vi "Rule_Check_Win.vi"(8 "error in":errorcluster, 9 "Exact Five":bool, 10 "Last Move":T2={"Row"=7, "Col"=7, "Stone"=enum."Black"}, 11 "Grid":enum8{"Empty", "Black", "White"}[][](array[ring])=[[enum."Empty", enum."Empty", enum."Empty", enum."Empty", enum."Empty", enum."Empty", enum."Empty", enum."Empty", enum."Empty", enum."Empty", enum."Empty", enum."Empty", enum."Empty", enum."Empty", enum."Empty"], [enum."Empty", enum."Empty", enum."Empty", enum."Empty", enum."Empty", enum."Empty", enum."Empty", enum."Empty", enum."Empty", enum."Empty", enum."Empty", enum."Empty", enum."Empty", enum."Empty", enum."Empty"], [enum."Empty", enum."Empty", enum."Empty", enum."Empty", enum."Empty", enum."Empty", enum."Empty", enum."Empty", enum."Empty", enum."Empty", enum."Empty", enum."Empty", enum."Empty", enum."Empty", enum."Empty"], [enum."Empty", enum."Empty", enum."Empty", enum."Empty", enum."Empty", enum."Empty", enum."Empty", enum."Empty", enum."Empty", enum."Empty", enum."Empty", enum."Empty", enum."Empty", enum."Empty", enum."Empty"], [enum."Empty", enum."Empty", enum."Empty", enum."Empty", enum."Empty", enum."Empty", enum."Empty", enum."Empty", enum."Empty", enum."Empty", enum."Empty", enum."Empty", enum."Empty", enum."Empty", enum."Empty"], [enum."Empty", enum."Empty", enum."Empty", enum."Empty", enum."Empty", enum."Empty", enum."Empty", enum."Empty", enum."Empty", enum."Empty", enum."Empty", enum."Empty", enum."Empty", enum."Empty", enum."Empty"], [enum."Empty", enum."Empty", enum."Empty", enum."Empty", enum."Empty", enum."Empty", enum."Empty", enum."Empty", enum."Empty", enum."Empty", enum."Empty", enum."Empty", enum."Empty", enum."Empty", enum."Empty"], [enum."Empty", enum."Empty", enum."Empty", enum."Empty", enum."Empty", enum."Empty", enum."Empty", enum."Empty", enum."Empty", enum."Empty", enum."Empty", enum."Empty", enum."Empty", enum."Empty", enum."Empty"], [enum."Empty", enum."Empty", enum."Empty", enum."Empty", enum."Empty", enum."Empty", enum."Empty", enum."Empty", enum."Empty", enum."Empty", enum."Empty", enum."Empty", enum."Empty", enum."Empty", enum."Empty"], [enum."Empty", enum."Empty", enum."Empty", enum."Empty", enum."Empty", enum."Empty", enum."Empty", enum."Empty", enum."Empty", enum."Empty", enum."Empty", enum."Empty", enum."Empty", enum."Empty", enum."Empty"], [enum."Empty", enum."Empty", enum."Empty", enum."Empty", enum."Empty", enum."Empty", enum."Empty", enum."Empty", enum."Empty", enum."Empty", enum."Empty", enum."Empty", enum."Empty", enum."Empty", enum."Empty"], [enum."Empty", enum."Empty", enum."Empty", enum."Empty", enum."Empty", enum."Empty", enum."Empty", enum."Empty", enum."Empty", enum."Empty", enum."Empty", enum."Empty", enum."Empty", enum."Empty", enum."Empty"], [enum."Empty", enum."Empty", enum."Empty", enum."Empty", enum."Empty", enum."Empty", enum."Empty", enum."Empty", enum."Empty", enum."Empty", enum."Empty", enum."Empty", enum."Empty", enum."Empty", enum."Empty"], [enum."Empty", enum."Empty", enum."Empty", enum."Empty", enum."Empty", enum."Empty", enum."Empty", enum."Empty", enum."Empty", enum."Empty", enum."Empty", enum."Empty", enum."Empty", enum."Empty", enum."Empty"], [enum."Empty", enum."Empty", enum."Empty", enum."Empty", enum."Empty", enum."Empty", enum."Empty", enum."Empty", enum."Empty", enum."Empty", enum."Empty", enum."Empty", enum."Empty", enum."Empty", enum."Empty"]]) -> (0 "error out":errorcluster, 1 "Run Length":i32, 2 "Win Line":T1(array[cluster]), 3 "Win?":bool)   [LabVIEW 2026]
doc: "마지막 착수 위치에서 4방향으로 연속 돌을 세어 5목 여부를 판정한다.\nExact Five=True(렌주룰 흑)이면 정확히 5개만 승리, False면 5개 이상 승리.\nWin Line = 승리한 방향의 5칸 좌표, Run Length = 4방향 중 가장 긴 연속 수."
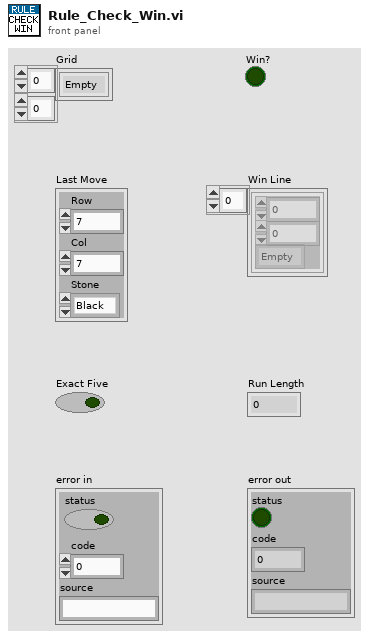
[diagram p1: front panel]
types:
  T1 = cluster{"Row":i32, "Col":i32, "Stone":enum8{"Empty", "Black", "White"}}[]
  T2 = cluster{"Row":i32, "Col":i32, "Stone":enum8{"Empty", "Black", "White"}}
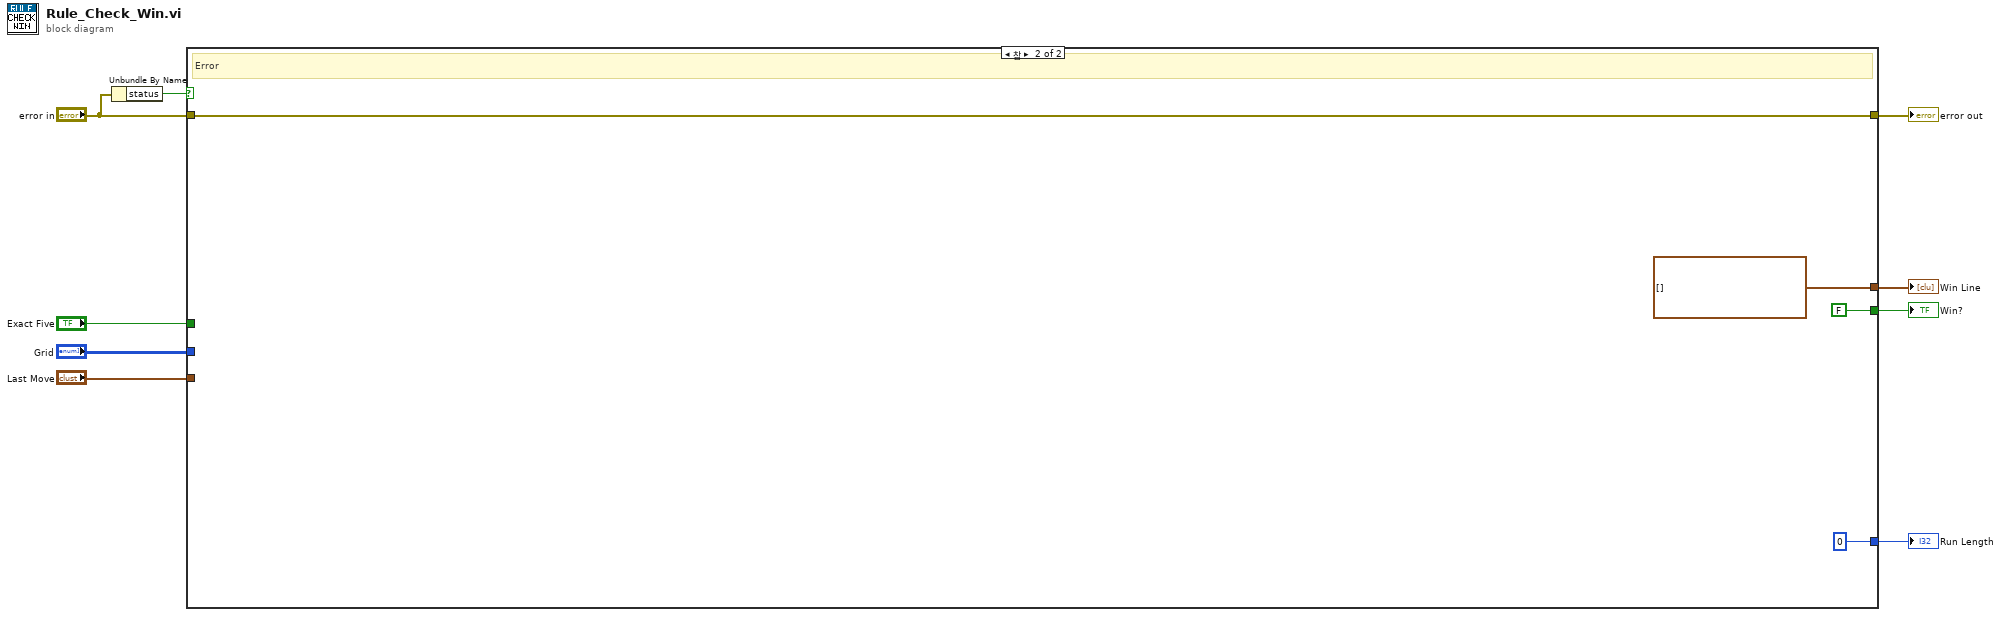
[diagram p0: block diagram]
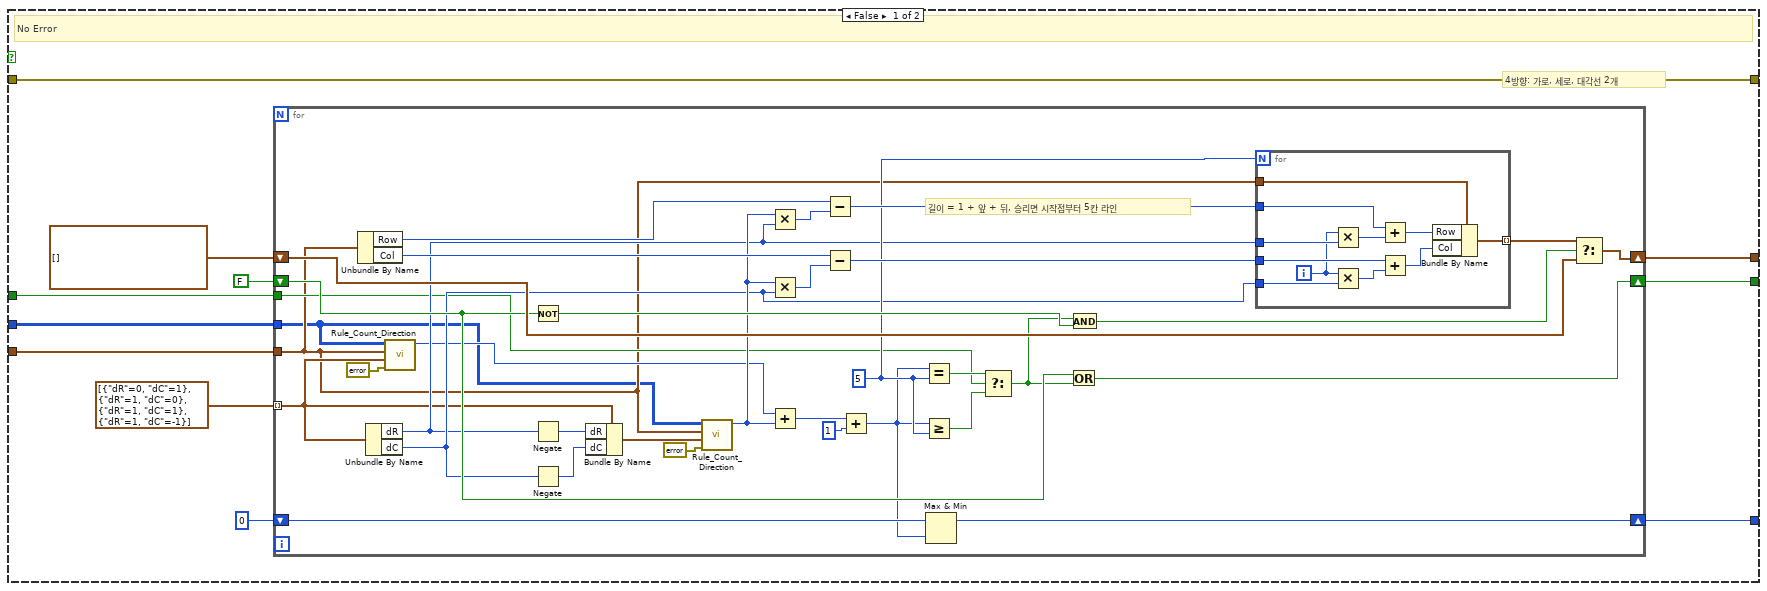
[diagram p2: hidden frame]
diagram:
  n1 = Unbundle By Name("error in") -> ("status"=w5:bool)
  n2 = case shown="참" w5 {
    tunnel: "Grid" -> [w10 _]
    tunnel: "Last Move" -> [w11 _]
    tunnel: "Exact Five" -> [w12 _]
    tunnel: "error in" -> [w13 w67]
    tunnel: [w18 FALSE] -> w6
    tunnel: [w19 T1 []] -> w7
    tunnel: [w20 0] -> w8
    tunnel: [w13 w67] -> w9
    frame False {
      # "4방향: 가로, 세로, 대각선 2개"
      # "No Error"
      n3 = for {
        tunnel: cluster{"dR":i32, "dC":i32}[] [{"dR"=0, "dC"=1}, {"dR"=1, "dC"=0}, {"dR"=1, "dC"=1}, {"dR"=1, "dC"=-1}] ("Directions") -> [w24] mode=indexing
        shift-right: [w53] -> w18
        shift-left: FALSE -> [w49]
        shift-right: [w51] -> w19
        shift-left: T1 [] -> [w52]
        shift-right: [w54] -> w20
        shift-left: 0 -> [w55]
        tunnel: w10 -> [w21]
        tunnel: w11 -> [w22]
        tunnel: w12 -> [w23]
        w37 = 5
        # "길이 = 1 + 앞 + 뒤, 승리면 시작점부터 5칸 라인"
        n4 = Unbundle By Name(w22) -> ("Row"=w41:i32, "Col"=w42:i32)
        n5 = Unbundle By Name(w24) -> ("dR"=w27:i32, "dC"=w28:i32)
        n6 = call "Rule_Count_Direction.vi"("error in"=errorcluster {"status"=FALSE, "code"=0, "source"=""}, "Direction"=w24, "Move"=w22, "Grid"=w21) -> ("Count"=w26:i32)  [unwired: 5 in, 2 out]
        n7 = Not(x=w49) -> (.not. x?=w48:bool)
        n8 = Negate(x=w27) -> (-x=w29:i32)
        n9 = Negate(x=w28) -> (-x=w30:i32)
        n10 = Bundle By Name(cluster=w24, "dR"=w29, "dC"=w30) -> (w31:cluster{"dR":i32, "dC":i32})
        n11 = call "Rule_Count_Direction.vi"("error in"=errorcluster {"status"=FALSE, "code"=0, "source"=""}, "Direction"=w31, "Move"=w22, "Grid"=w21) -> ("Count"=w33:i32)  [unwired: 5 in, 2 out]
        n12 = Multiply(x=w33, y=w27) -> (x*y=w43:i32)
        n13 = Multiply(x=w33, y=w28) -> (x*y=w45:i32)
        n14 = Add(x=w26, y=w33) -> (x+y=w34:i32)
        n15 = Subtract(x=w41, y=w43) -> (x-y=w44:i32)
        n16 = Subtract(x=w42, y=w45) -> (x-y=w46:i32)
        n17 = Add(x=w34, y=1) -> (x+y=w36:i32)
        n18 = Equal?(x=w36, y=w37) -> (x = y?=w38:bool)
        n19 = Greater Or Equal?(x=w36, y=w37) -> (x >= y?=w39:bool)
        n20 = Max & Min(x=w55, y=w36) -> (max(x,y)=w54:i32)  [unwired: 1 out]
        n21 = Select(t=w38, s=w23, f=w39) -> (s? t:f=w40:bool)
        n22 = Or(x=w49, y=w40) -> (x .or. y?=w53:bool)
        n23 = And(x=w40, y=w48) -> (x .and. y?=w50:bool)
        n24 = for {
          N: w37 -> [_]
          tunnel: w27 -> [w59]
          tunnel: w28 -> [w60]
          tunnel: w22 -> [w61]
          tunnel: w44 -> [w57]
          tunnel: w46 -> [w58]
          tunnel: [w66] -> w47 mode=indexing
          i -> [w56]
          n25 = Multiply(x=w56, y=w59) -> (x*y=w62:i32)
          n26 = Multiply(x=w56, y=w60) -> (x*y=w64:i32)
          n27 = Add(x=w57, y=w62) -> (x+y=w63:i32)
          n28 = Add(x=w58, y=w64) -> (x+y=w65:i32)
          n29 = Bundle By Name(cluster=w61, "Row"=w63, "Col"=w65) -> (w66:T2)
        }
        n30 = Select(t=w47, s=w50, f=w52) -> (s? t:f=w51:T1)
      }
    }
    frame True {
      # "Error"
    }
  }
  "Win?" <- w6
  "Win Line" <- w7
  "Run Length" <- w8
  "error out" <- w9
